vi "RespondUnauth.vi"(8 "error in (no error)":errorcluster, 11 "LabVIEW Web Service Request":refnum<class "Web Request.lvclass"> caption="LabVIEW Web Service Request in") -> (0 "error out":errorcluster)   [LabVIEW 2017]
uses:
  <vilib>/wsapi/Web Request.lvclass
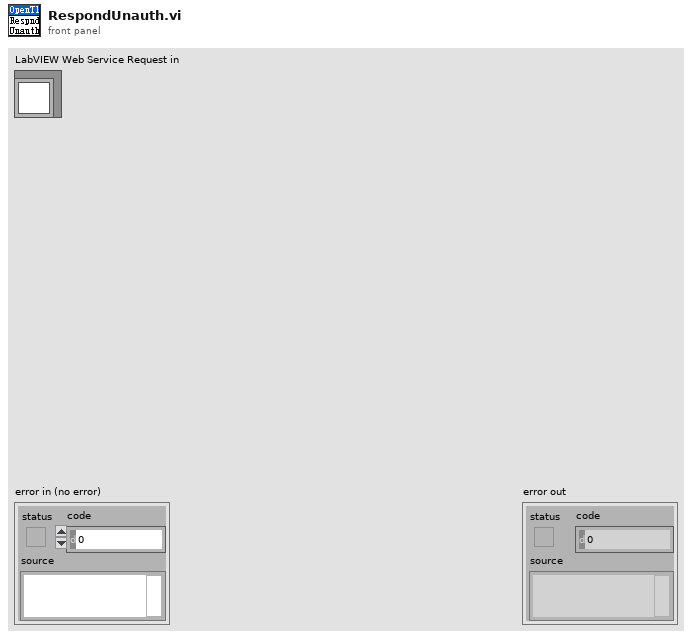
[diagram p1: front panel]
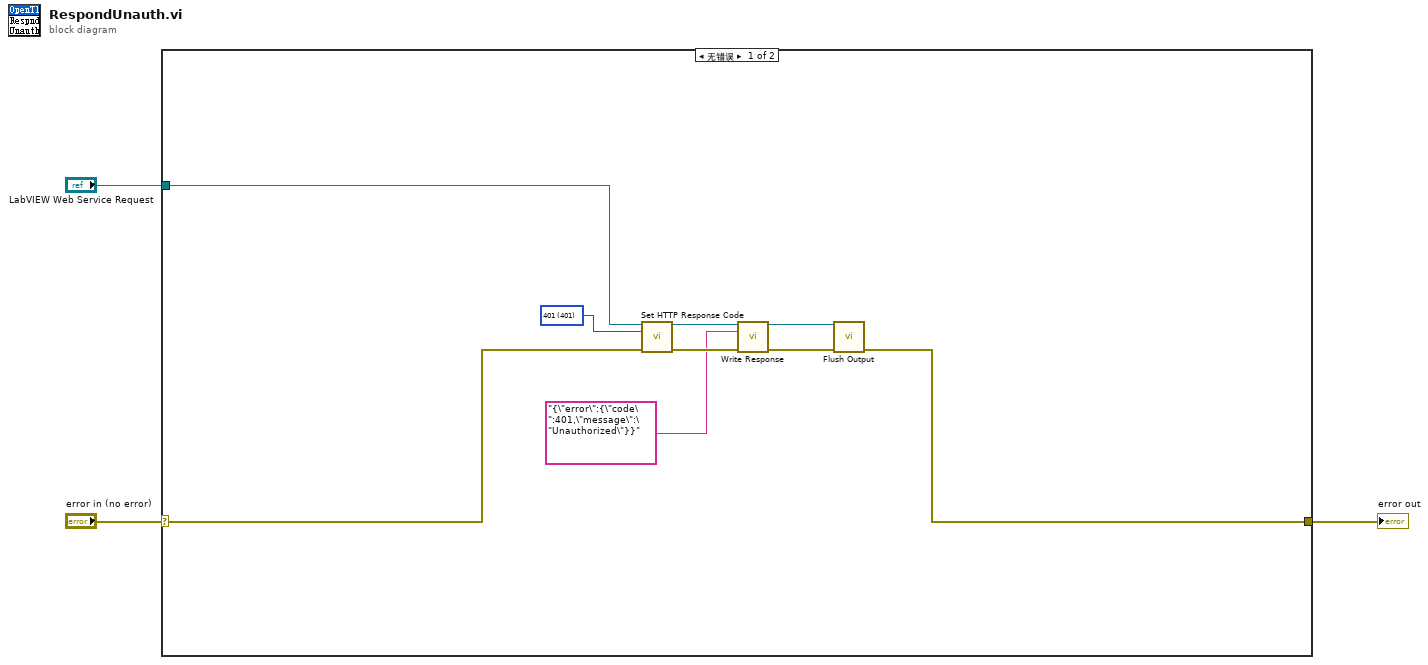
[diagram p0: block diagram]
diagram:
  n1 = case shown="无错误" "error in (no error)" {
    selector: "error in (no error)" -> [w6 w13]
    tunnel: [w4 w13] -> w2
    tunnel: "LabVIEW Web Service Request" -> [w5 _]
    frame No Error {
      w12 = 401 items=["100"=100, "101"=101, "200"=200, "201"=201, "202"=202, "203"=203, "204"=204, "205"=205, "206"=206, "300"=300, "301"=301, "302"=302, "303"=303, "304"=304, "305"=305, "306"=306, "307"=307, "400"=400, "401"=401, "402"=402, "403"=403, "404"=404, "405"=405, "406"=406, "407"=407, "408"=408, "409"=409, "410"=410, "411"=411, "412"=412, "413"=413, "414"=414, "415"=415, "416"=416, "417"=417, "500"=500, "501"=501, "502"=502, "503"=503, "504"=504, "505"=505] ("response code (200)")
      n2 = call <vilib>:"Set HTTP Response Code.vi"("LabVIEW Web Service Request"=w5, "response code (200)"=w12, "error in (no error)"=w6) -> ("LabVIEW Web Service Request out"=w8:refnum<class "Web Request.lvclass">, "error out"=w9:errorcluster)  [unwired: 11 in]
      n3 = call <vilib>:"Write Response.vi"("LabVIEW Web Service Request"=w8, "response string"="{\"error\":{\"code\":401,\"message\":\"Unauthorized\"}}", "error in (no error)"=w9) -> ("LabVIEW Web Service Request out"=w10:refnum<class "Web Request.lvclass">, "error out"=w11:errorcluster)  [unwired: 11 in]
      n4 = call <vilib>:"Flush Output.vi"("LabVIEW Web Service Request"=w10, "error in (no error)"=w11) -> ("error out"=w4:errorcluster)  [unwired: 12 in, 1 out]
    }
    frame Error {
    }
  }
  "error out" <- w2
